vi "Quick Stacks.vi"(7 "Calling VI Ref":refnum<vi>) -> ()   [LabVIEW 2016]
uses:
  Hardware Configuration/Hardware Configuration Controls/Device Function.ctl
  Hardware Configuration/Hardware Configuration Controls/Device Type.ctl
  Quick Stacks Type Defs/Quick Stacks Notifier Type.ctl
  Quick Stacks Type Defs/Quick Stack Actions.ctl
  <vilib>/Utility/miscctls.llb/LVPointTypeDef.ctl
  Device Library/Stages/Stages Controls/Stage Actions.ctl
  Color Steps/Color Steps Type Def/Color Step Actions.ctl
  Tools/TIFF Image Read and Write/ImageJ TIF Type Defs/TIF Write Image Information.ctl
  Device Library/Cameras/Camera Controls/Generic Camera Actions.ctl
  Laser Control/Laser Power Control/Laser Power Control Type Defs/Laser Power Ctrl Messenger Actions.ctl
  shell32.dll
panel:
  in  "Camera 02":bool=TRUE
  in  "Camera 01":bool=TRUE
  out "Current Cycle":u16
  out "Current Step":u16
  in  "Start":bool
  in  "Number of Cycles":u16=1 min=1
  in  "Cycle Delay (s)":u32
  in  "Frames Per Step":u16=1 min=1
  in  "Base Save Path":path
  in  "File Name":string="Test Image"
  out "Z Range (µm)":dbl
  in  "Number of Steps":u16=1
  out "Step Size (µm)":dbl format="%#_3g"
  out "End Position (µm)":dbl
  out "Start Position (µm)":dbl
  in  "Set Z End":bool
  in  "Set Z Start":bool
  in  "Quit":bool
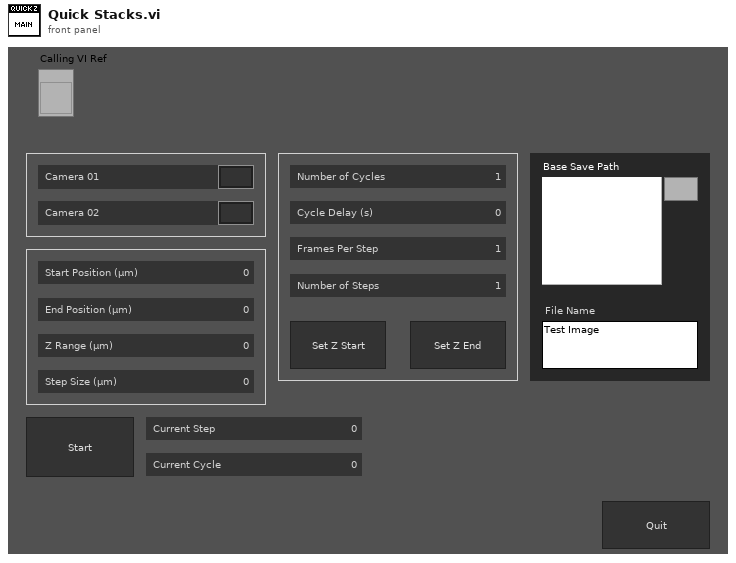
[diagram p1: front panel]
types:
  T1 = enum16{"Always On", "Always Off", "Off While Running"}
  T2 = typedef "LVPointTypeDef.ctl" = cluster{"Horizontal":i16, "Vertical":i16}
  T3 = typedef "Quick Stack Actions.ctl" = enum16{"Idle", "Update Range", "Start Acquisition", "Initial C Step", "Open File", "Close File", "Start Camera", "Stop Camera", "Laser On", "Laser Off", "Get Image", "Step Z", "Move to Z Start", "Step Color", "Check Cycle", "Abort", "Exit Loop", "Quit"}
  T4 = typedef "Quick Stacks Notifier Type.ctl" = cluster{"Actions":T3, "Start Z (µm)":dbl, "End Z (µm)":dbl, "Z Size (µm)":dbl, "Num of Steps":u16, "Frames per Step":u16, "Cycle Delay (s)":u32, "Num of Cycles":u16, "Save Path":path, "Running?":bool, "Save File Refs":refnum<file>[]}
  T5 = typedef "Device Function.ctl" = enum16{"Primary", "Secondary", "Overview", "Wide Field Drift Correction", "642 nm Excitation", "560 nm Excitation", "940 nm Excitation", "546 nm Excitation", "488 nm Excitation", "405 nm Excitation", "Objective Drift Correction", "4Pi Objective Lock", "Objective XY", "Objective Z", "Sample XY", "Sample Coarse Z", "Sample Z", "4Pi Lower", "4Pi Upper", "Mojo", "Adj Cavity", "Line Scanning", "Alert"}
  T6 = typedef "Device Type.ctl" = enum16{"AOTF", "Camera", "Deformable Mirror", "Laser", "Shutter", "Stage", "Waveform", "FPGA", "Email", "Filter Wheel"}
  T7 = typedef "LVRectTypeDef.ctl" = cluster{"Left":i16, "Top":i16, "Right":i16, "Bottom":i16}
  T8 = typedef "LVBoundsTypeDef.ctl" = cluster{"Width":u32, "Height":u32}
  T9 = typedef "Stage Actions.ctl" = enum16{"Get Position", "MVR", "MOVE", "HALT", "ONTARGET", "ERROR", "REFERENCE", "INIT", "VELOCITY", "STATUS", "EXIT", "HOME", "ZEROPOS", "NANOPOS", "ANALOG", "QUIT"}
  T10 = typedef "Color Step Actions.ctl" = enum16{"Add Step", "Update Step", "Remove Step", "Clear All", "Get Status", "Next Step", "Go To Step", "Save Preset", "Change Preset", "Update Names", "Quit"}
  T11 = typedef "Generic Camera Actions.ctl" = enum16{"Status", "Live Preview", "Capture", "Abort", "Set Exposure Time (s)", "Get Exposure Time (s)", "Record Settings", "Set ROI", "Get ROI", "Defect Correction On/Off", "Cooler On/Off", "Fan On/Off", "Quti"}
  T12 = typedef "TIF Write Image Information.ctl" = cluster{"Image Width (Pixels)":u32, "Image Height (Pixels)":u32, "Pixel Width (µm)":dbl, "Pixel Height (µm)":dbl, "Bits Per Sample (e.g. 16)":u32, "No. of Frames":u32, "No. of Slices":u32, "Time Step (sec)":dbl, "Z Step (µm)":dbl}
  T13 = typedef "Laser Power Ctrl Messenger Actions.ctl" = enum16{"All Active On", "All Off", "Adjust Power", "Line On/Off", "Get Status"}
  T14 = typedef "IMAQ Image.ctl" = refnum<image>
  T15 = typedef "Camera IMAQ Key Info.ctl" = cluster{"Frame":u32, "Sensor Height":i32, "Sensor Width":i32, "ROI Height":i32, "ROI Width":i32, "ROI Enable?":bool, "Bit per Pixel":u8}
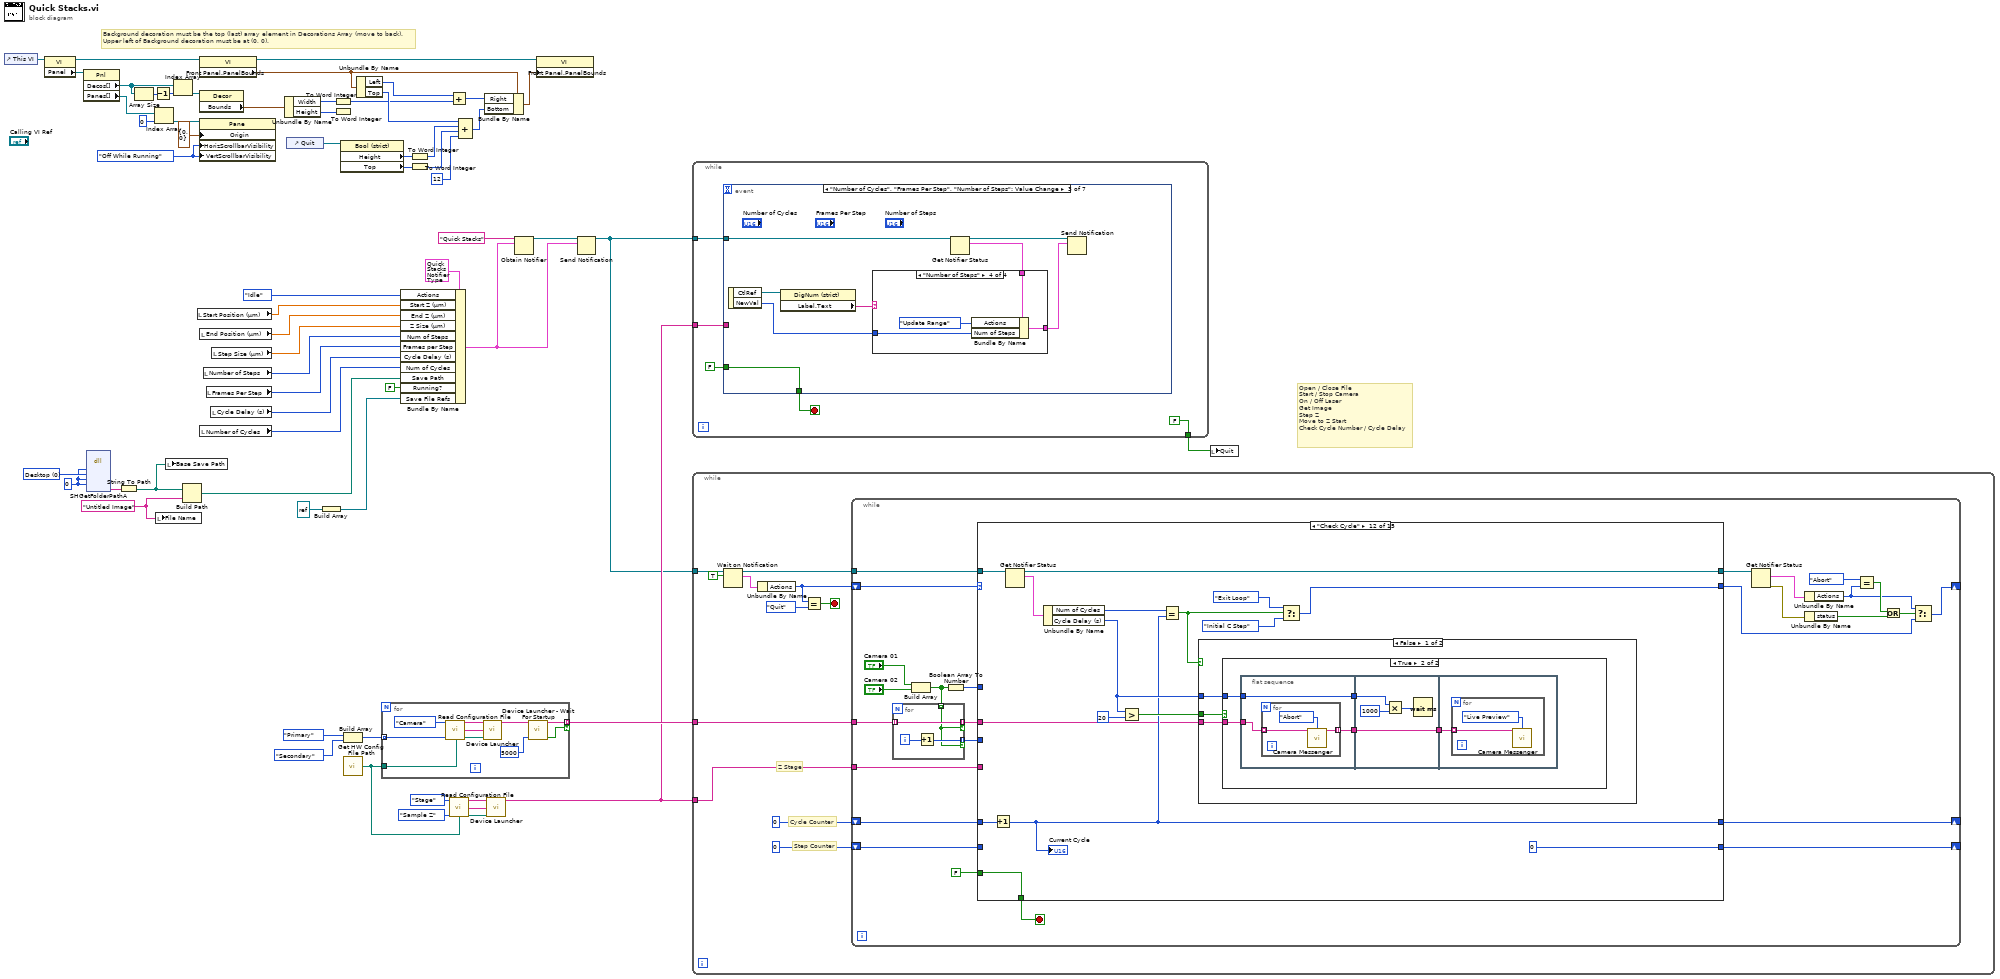
[diagram p0: block diagram]
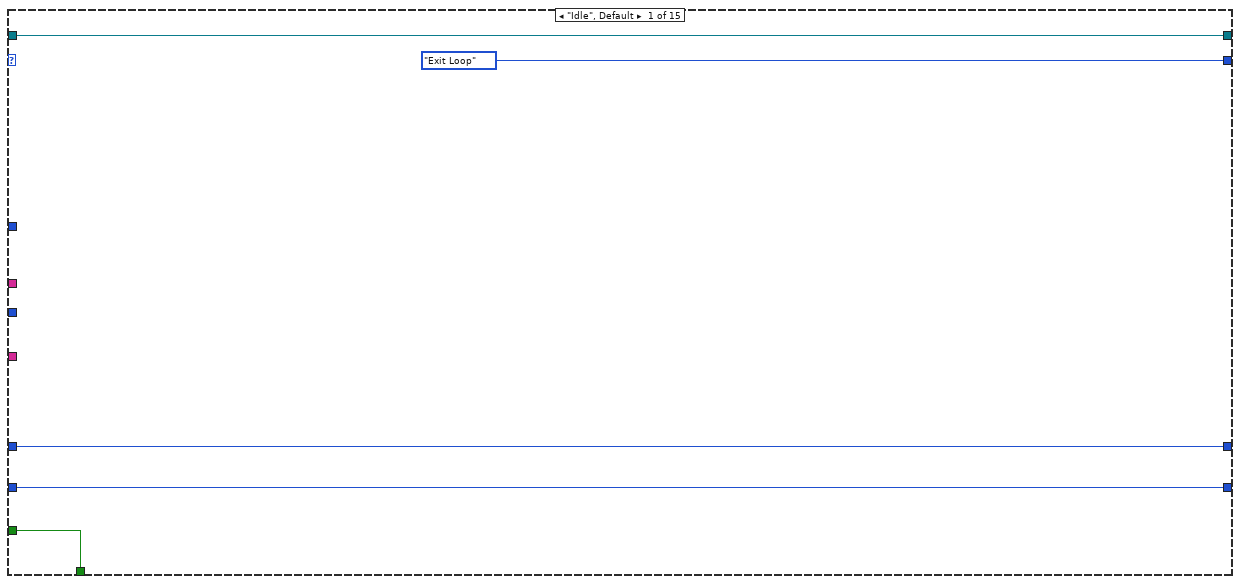
[diagram p2: hidden frame]
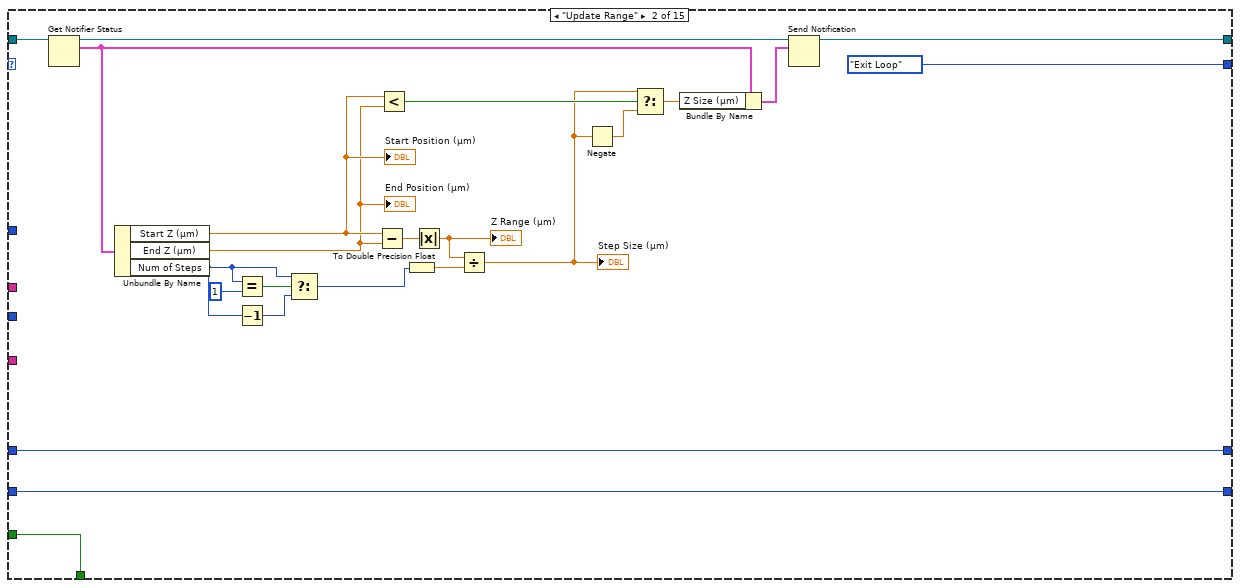
[diagram p3: hidden frame]
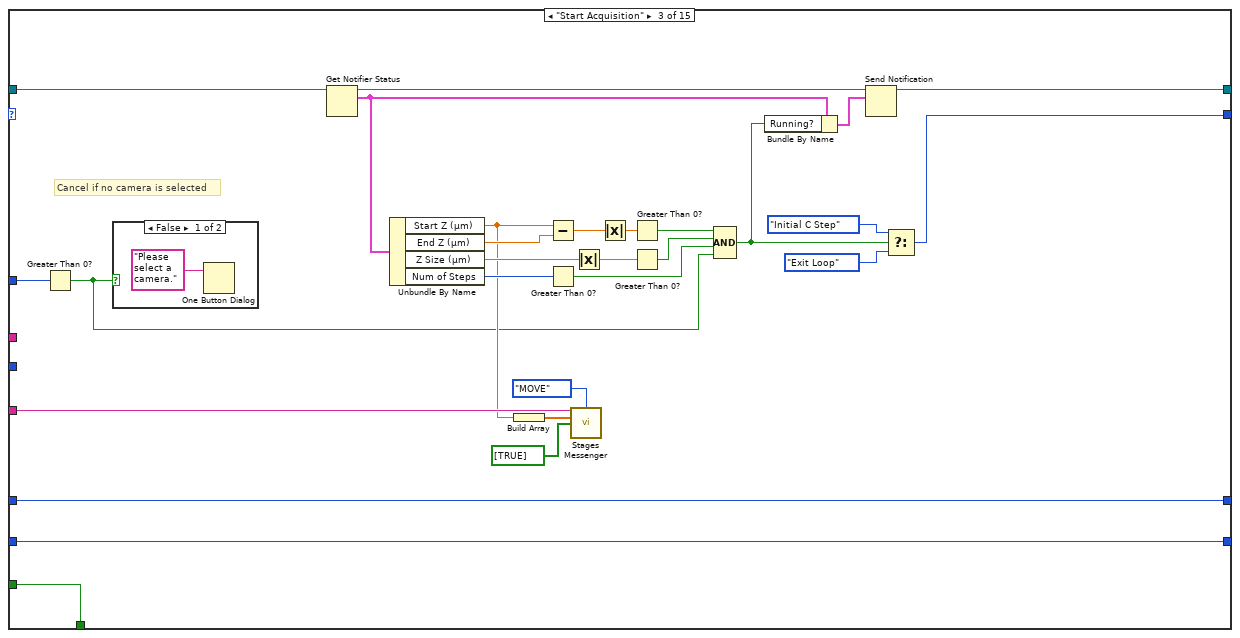
[diagram p4: hidden frame]
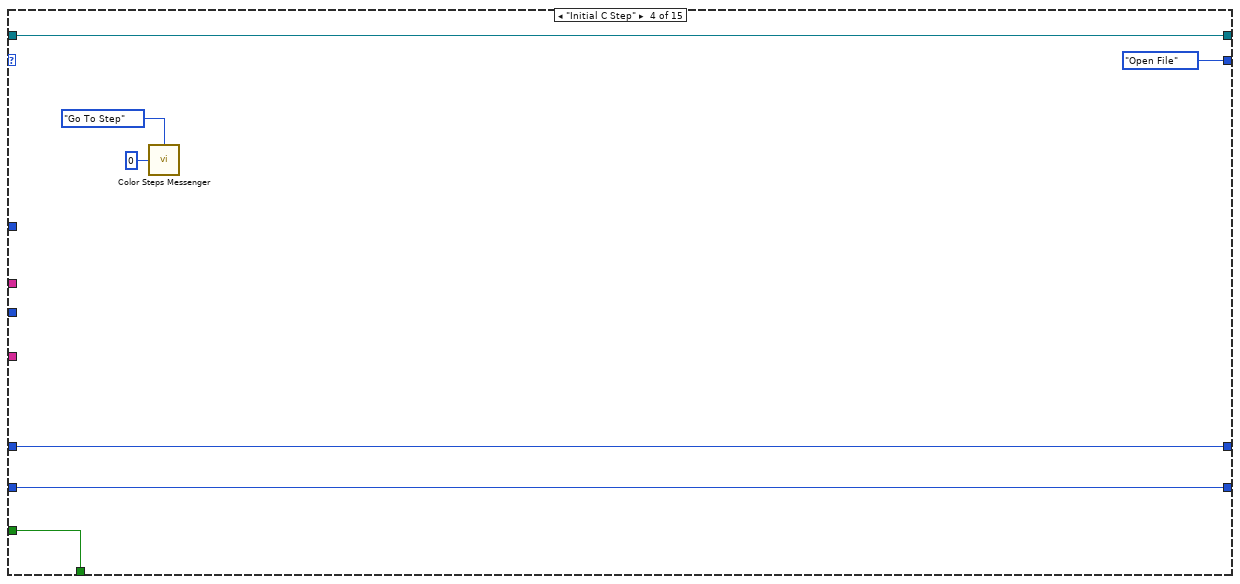
[diagram p6: hidden frame]
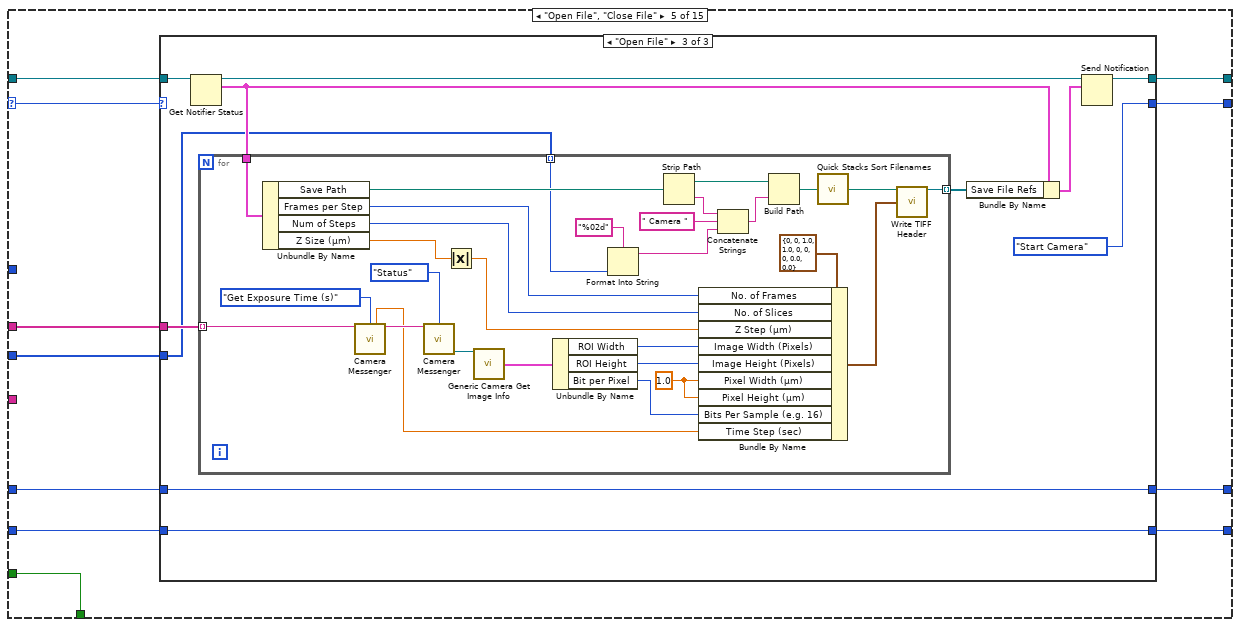
[diagram p7: hidden frame]
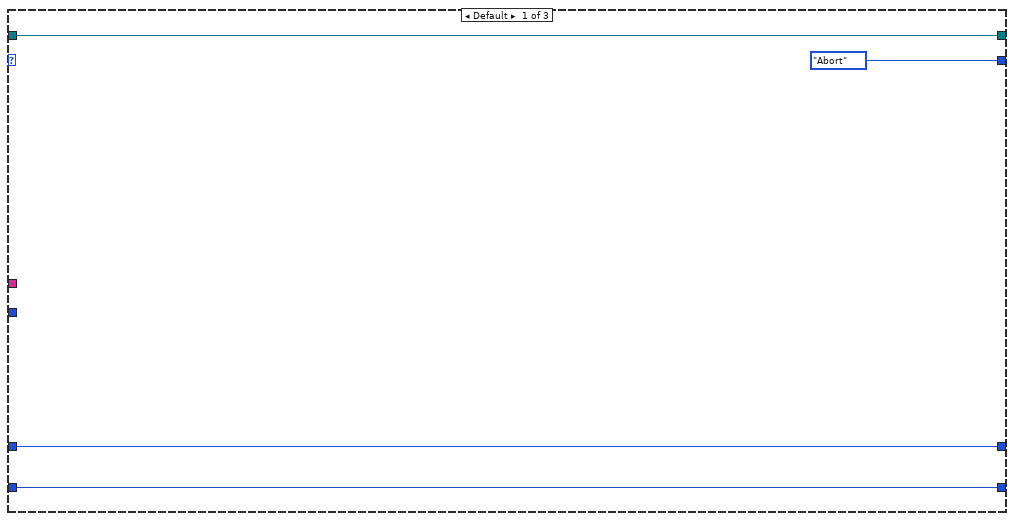
[diagram p8: hidden frame]
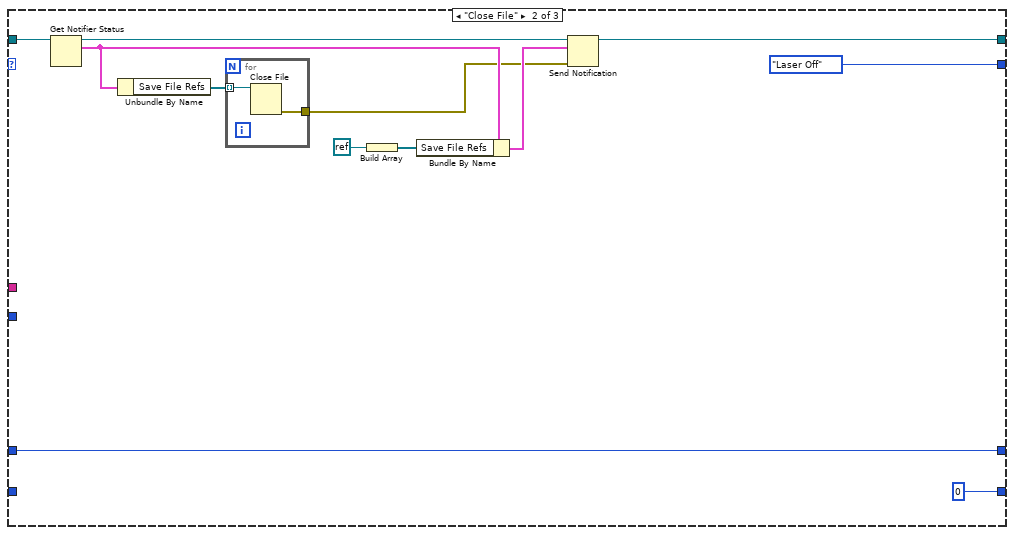
[diagram p9: hidden frame]
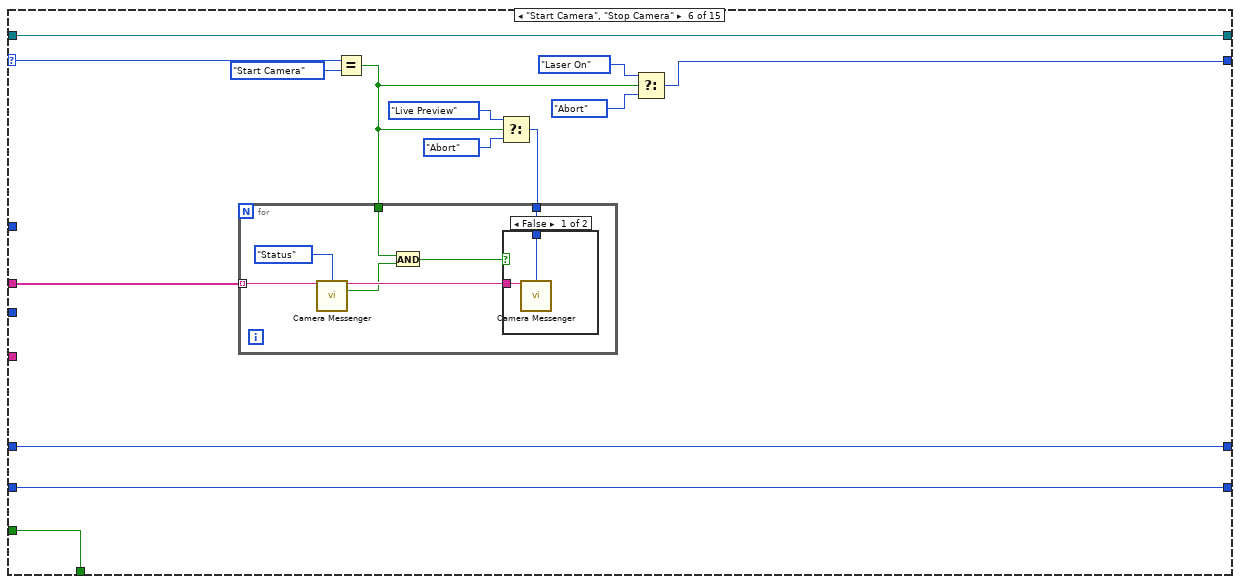
[diagram p10: hidden frame]
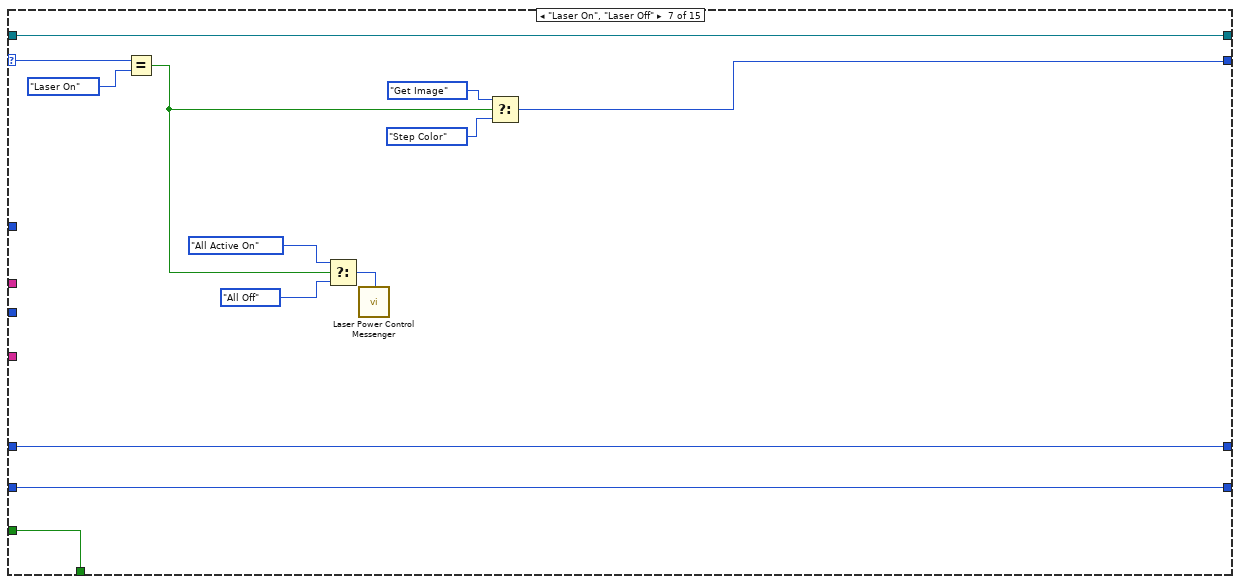
[diagram p12: hidden frame]
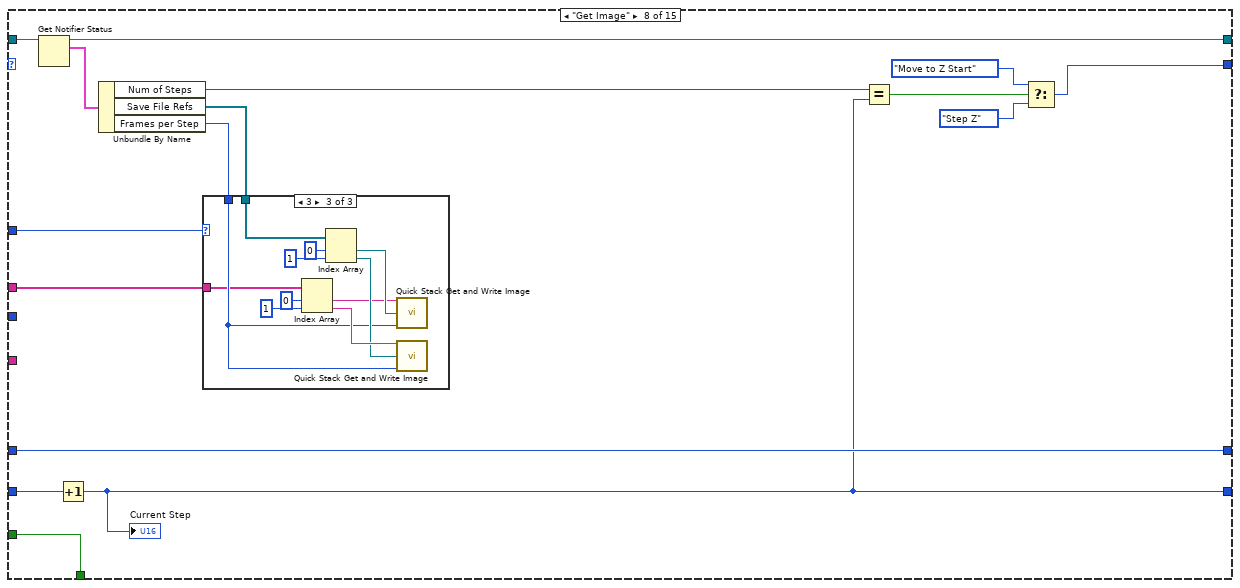
[diagram p13: hidden frame]
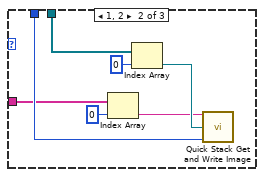
[diagram p15: hidden frame]
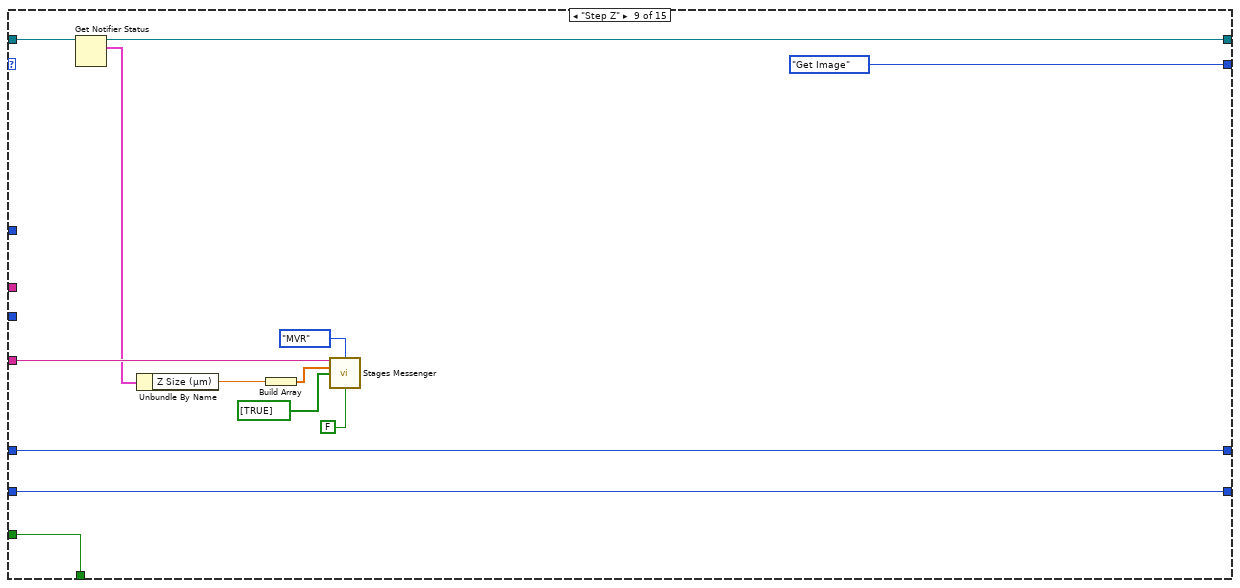
[diagram p16: hidden frame]
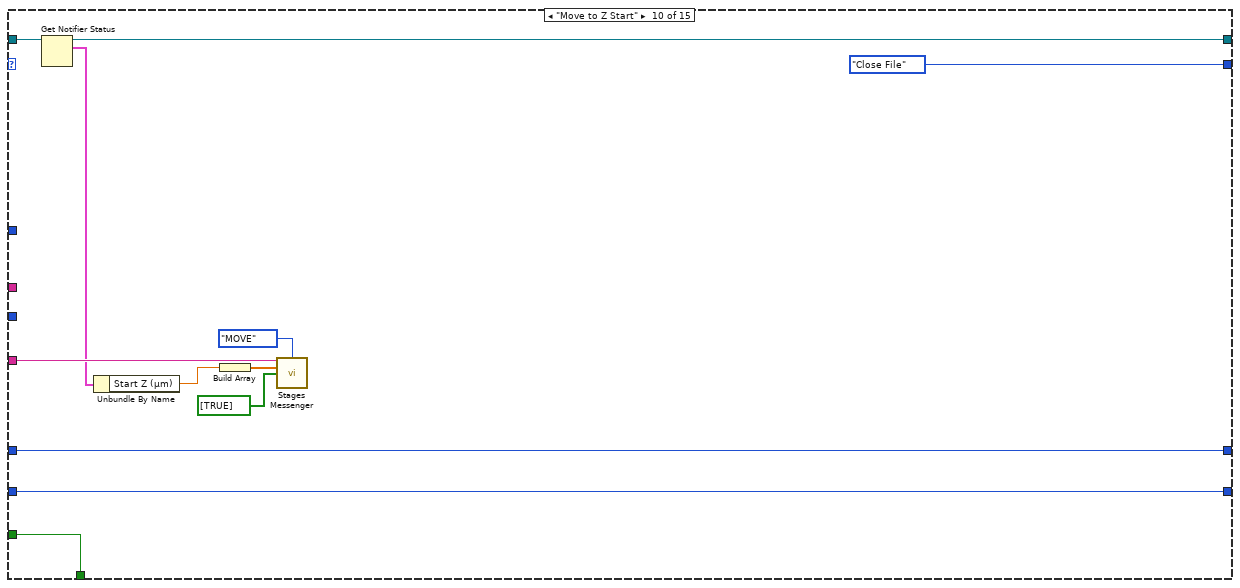
[diagram p17: hidden frame]
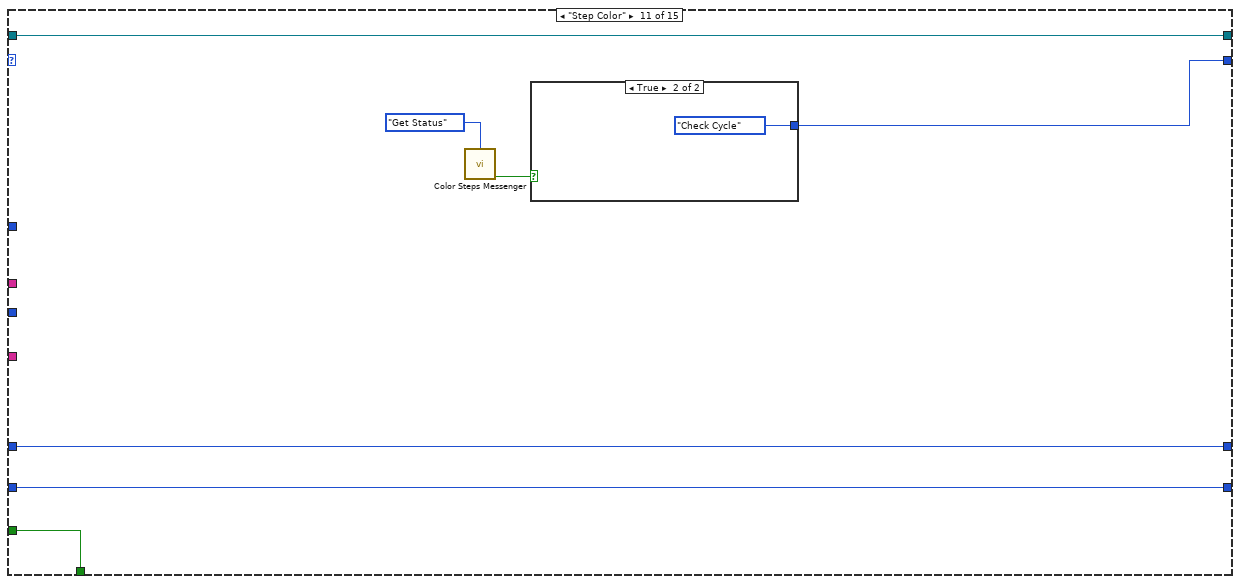
[diagram p18: hidden frame]
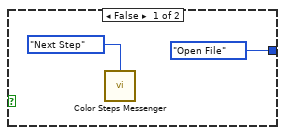
[diagram p19: hidden frame]
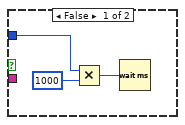
[diagram p20: hidden frame]
diagram:
  w15 = T1."Off While Running" ("Vertical Scrollbar Visibility")
  w49 = "Untitled Image"
  w52 = 0 items=["Desktop"=0, "Personal Documents"=5, "AppData"=26, "Local AppData"=28, "Common AppData"=35, "Program Files"=38, "Program Files Common"=43, "Common Documents"=46] ("Requested Path")
  w51 = 0 ("HWND")
  # "Background decoration must be the top (last) array element in Decorations Array (move to back).\nUpper left of Background decoration must be at (0, 0)."
  # "Open / Close File\nStart / Stop Camera\nOn / Off Laser\nGet Image\nStep Z\nMove to Z Start\nCheck Cycle Number / Cycle Delay"
  n1 = control-ref of="This VI"() -> (w7:refnum<vi>)
  n2 = property class="VI"(reference=w7) -> (reference out=w16:refnum<vi>, "Panel"=w8:refnum<vi>)  [unwired: 1 in, 1 out]
  n3 = property class="Pnl"(reference=w8) -> ("Decos[]"=w6:refnum<vi>[], "Panes[]"=w12:refnum<vi>[])  [unwired: 1 in, 2 out]
  n4 = dll-call lib="shell32.dll" fn="SHGetFolderPathA"("HWND"=w51, "nFolder"=w52, "hToken"=w51, "dwFlags"=w51) -> ("pszPath"=w50:string)  [unwired: 9 in, 2 out]
  n5 = String To Path(string=w50) -> (path=w48:path)
  n6 = Array Size(array=w6) -> (size(s)=w4:i32)
  n7 = Decrement(x=w4) -> (x-1=w5:i32)
  n8 = Index Array(array=w12, index=0) -> (element=w11:refnum<vi>)
  n9 = local write "File Name"(w49) -> ()
  n10 = local write "Base Save Path"(w48) -> ()
  n11 = Index Array(array=w6, index=w5) -> (element=w14:refnum<vi>)
  n12 = Build Path(base path=w48, name or relative path=w49) -> (appended path=w38:path)
  n13 = local read "Start Position (µm)"() -> (w39:dbl)
  n14 = property class="VI"(reference=w16) -> (reference out=w18:refnum<vi>, "Front Panel.PanelBounds"=w19:T7)  [unwired: 1 in, 1 out]
  n15 = property class="Decor"(reference=w14) -> ("Bounds"=w17:T8)  [unwired: 1 in, 2 out]
  n16 = property class="Pane"(reference=w11, "Origin"=T2 {"Horizontal"=0, "Vertical"=0}, "HorizScrollbarVisibility"=w15, "VertScrollbarVisibility"=w15) -> ()  [unwired: 1 in, 2 out]
  n17 = local read "End Position (µm)"() -> (w40:dbl)
  n18 = local read "Number of Cycles"() -> (w45:u16)
  n19 = local read "Number of Steps"() -> (w42:u16)
  n20 = local read "Frames Per Step"() -> (w43:u16)
  n21 = local read "Cycle Delay (s)"() -> (w44:u32)
  n22 = local read "Step Size (µm)"() -> (w41:dbl)
  n23 = Unbundle By Name(w17) -> ("Width"=w22:u32, "Height"=w25:u32)
  n24 = control-ref of="Quit"() -> (w9:refnum<vi>)
  n25 = Build Array(refnum<file> refnum ("Save File Ref")) -> (w1:refnum<file>[])
  n26 = To Word Integer(number=w22) -> (16bit integer=w24:i16)
  n27 = To Word Integer(number=w25) -> ()  [unwired: 1 out]
  n28 = property class="Bool (strict)"(reference=w9) -> ("Height"=w27:u32, "Top"=w28:i32)  [unwired: 1 in, 2 out]
  n29 = Build Array(Device_Function."Primary" ("Device Function"), Device_Function."Secondary" ("Device Function")) -> (w61:T5[])
  n30 = call "Get HW Config File Path.vi"() -> ("File Path"=w53:path)  [unwired: 14 in, 1 out]
  n31 = Unbundle By Name(w19) -> ("Left"=w21:i16, "Top"=w32:i16)
  n32 = for {
    tunnel: w61 -> [w69] mode=indexing
    tunnel: w53 -> [w68]
    tunnel: [w66] -> w54 mode=indexing if=w65
    n33 = call "Read Configuration File.vi"("Device Type"=Device_Type."Camera", "Device Function"=w69, "Config File Path"=w68) -> ("Unique Notifier Name"=w71:string, "Device Ports/IDs/Channels"=w73:string[], "Device Engine Path"=w72:path)  [unwired: 9 in, 1 out]
    n34 = call "Device Launcher.vi"("Notifier Name"=w71, "Device Ports/IDs/Channels"=w73, "Device Engine Path"=w72) -> ("Notifier Name"=w67:string)  [unwired: 11 in, 1 out]
    n35 = call "Device Launcher - Wait For Startup.vi"("Notifier Name"=w67, "Wait Time (ms)"=5000) -> ("Notifier Name (Dup)"=w66:string, "Running?"=w65:bool)  [unwired: 12 in]
  }
  n36 = Bundle By Name(cluster=T4 {"Actions"=enum."Idle", "Start Z (µm)"=0.0, "End Z (µm)"=0.0, "Z Size (µm)"=0.0, "Num of Steps"=0, "Frames per Step"=0, "Cycle Delay (s)"=0, "Num of Cycles"=0, "Save Path"=path "", "Running?"=FALSE, "Save File Refs"=[]} ("Stack Parameters"), "Actions"=Quick_Stack_Actions."Idle", "Start Z (µm)"=w39, "End Z (µm)"=w40, "Z Size (µm)"=w41, "Num of Steps"=w42, "Frames per Step"=w43, "Cycle Delay (s)"=w44, "Num of Cycles"=w45, "Save Path"=w38, "Running?"=FALSE ("Running"), "Save File Refs"=w1) -> (w33:T4)
  n37 = To Word Integer(number=w27) -> (16bit integer=w30:i16)
  n38 = To Word Integer(number=w28) -> (16bit integer=w31:i16)
  n39 = call "Read Configuration File.vi"("Device Type"=Device_Type."Stage", "Device Function"=Device_Function."Sample Z", "Config File Path"=w53) -> ("Unique Notifier Name"=w56:string, "Device Ports/IDs/Channels"=w58:string[], "Device Engine Path"=w57:path)  [unwired: 9 in, 1 out]
  n40 = Add(x=w21, y=w24) -> (x+y=w23:i16)
  n41 = Compound Arithmetic op=ADD(w32, w30, w31, i16 12 ("y")) -> (w26:i16)
  n42 = Bundle By Name(cluster=w19, "Right"=w23, "Bottom"=w26) -> (w20:T7)
  n43 = call "Device Launcher.vi"("Notifier Name"=w56, "Device Ports/IDs/Channels"=w58, "Device Engine Path"=w57) -> ("Notifier Name"=w37:string)  [unwired: 11 in, 1 out]
  n44 = Obtain Notifier(name (unnamed)="Quick Stacks", notification data type=w33) -> (notifier out=w35:refnum<notifier>)  [unwired: 2 in, 2 out]
  n45 = property class="VI"(reference=w18, "Front Panel.PanelBounds"=w20) -> ()  [unwired: 1 in, 2 out]
  n46 = Send Notification(notification=w33, notifier=w35) -> (notifier out=w34:refnum<notifier>)  [unwired: 1 in, 1 out]
  n47 = while {
    tunnel: w34 -> [w84]
    tunnel: w54 -> [w74]
    tunnel: w37 -> [w77]
    stop <- w81 stop-if-true
    # "Z Stage"
    # "Step Counter"
    # "Cycle Counter"
    n48 = Wait on Notification(notifier=w84, ignore previous (F)=TRUE) -> (notifier out=w80:refnum<notifier>, notification=w79:T4)  [unwired: 2 in, 2 out]
    n49 = Unbundle By Name(w79) -> ("Actions"=w78:T3)
    n50 = Equal?(x=w78, y=Quick_Stack_Actions."Quit") -> (x = y?=w81:bool)
    n51 = while {
      tunnel: w80 -> [w110]
      shift-right: [w92] -> _
      shift-left: w78 -> [w109]
      tunnel: w77 -> [w106]
      shift-right: [w102] -> _
      shift-left: u16 0 -> [w105]
      shift-right: [w103] -> _
      shift-left: u16 0 -> [w104]
      tunnel: w74 -> [w88]
      stop <- w107 stop-if-true
      n52 = Build Array("Camera 01", "Camera 02") -> (w87:bool[])
      n53 = for {
        tunnel: w88 -> [w431] mode=indexing
        tunnel: [w431] -> w89 mode=indexing if=w428
        tunnel: w87 -> [w428] mode=indexing
        tunnel: [w429] -> w85 mode=indexing if=w428
        i -> [w430]
        n54 = Increment(x=w430) -> (x+1=w429:i32)
      }
      n55 = Boolean Array To Number(Boolean array=w87) -> (number=w86:u32)
      n56 = case shown="\"Check Cycle\"" w109 {
        selector: w109 -> [_ _ _ _ w183 w256 w278 _ _ _ _ _ _ _ _]
        tunnel: w110 -> [w113 w136 w165 w174 w184 w249 w271 w293 w325 w333 w344 w361 w406 w417 w423]
        tunnel: FALSE -> [w115 w137 w166 w172 w185 w257 w279 w295 w326 w335 w345 w364 w407 _ _]
        tunnel: [w115 w137 w166 w172 w185 w257 w279 w295 w326 w335 w345 w364 w407 TRUE TRUE] -> w107
        tunnel: [Quick_Stack_Actions."Exit Loop" ("y") Quick_Stack_Actions."Exit Loop" ("y") w154 Quick_Stack_Actions."Open File" ("y") w182 w250 w275 w287 Quick_Stack_Actions."Get Image" ("y") Quick_Stack_Actions."Close File" ("y") w339 w355 Quick_Stack_Actions."Exit Loop" ("y") Quick_Stack_Actions."Exit Loop" ("y") Quick_Stack_Actions."Quit" ("y")] -> w93
        tunnel: w106 -> [_ _ w151 _ _ _ _ _ w323 w334 _ _ w401 _ _]
        tunnel: w105 -> [w112 w122 w147 w171 w178 w248 w273 w290 w322 w329 w341 w363 _ w420 w425]
        tunnel: w104 -> [w111 w121 w146 w170 w176 w247 w272 w294 w321 w330 w340 _ _ w419 w424]
        tunnel: [w113 w123 w144 w174 w181 w249 w271 w291 w320 w328 w344 w359 w398 w415 w423] -> w101
        tunnel: [w111 w121 w146 w170 w175 w247 w272 w284 w321 w330 w340 u16 0 w400 w419 w424] -> w103
        tunnel: [w112 w122 w147 w171 w177 w248 w273 w290 w322 w329 w341 w350 w400 w420 w425] -> w102
        tunnel: w89 -> [_ _ _ _ w180 w244 _ w281 _ _ _ w349 w394 _ _]
        tunnel: w86 -> [_ _ w140 _ _ _ _ w280 _ _ _ _ _ _ _]
        tunnel: w85 -> [_ _ _ _ w179 _ _ _ _ _ _ _ _ _ _]
        frame "Idle", Default {
        }
        frame "Update Range" {
          n57 = Get Notifier Status(notifier=w136) -> (notifier out=w135:refnum<notifier>, current notification=w134:T4)  [unwired: 1 in, 3 out]
          n58 = Unbundle By Name(w134) -> ("Start Z (µm)"=w130:dbl, "End Z (µm)"=w129:dbl, "Num of Steps"=w132:u16)
          "Start Position (µm)" <- w130
          "End Position (µm)" <- w129
          n59 = Equal?(x=w132, y=u16 1) -> (x = y?=w117:bool)
          n60 = Decrement(x=w132) -> (x-1=w118:u16)
          n61 = Select(t=w132, s=w117, f=w118) -> (s? t:f=w119:u16)
          n62 = Subtract(x=w130, y=w129) -> (x-y=w133:dbl)
          n63 = Less?(x=w130, y=w129) -> (x < y?=w127:bool)
          n64 = To Double Precision Float(number=w119) -> (double precision float=w120:dbl)
          n65 = Absolute Value(x=w133) -> (abs(x)=w131:dbl)
          "Z Range (µm)" <- w131
          n66 = Divide(x=w131, y=w120) -> (x/y=w125:dbl)
          "Step Size (µm)" <- w125
          n67 = Negate(x=w125) -> (-x=w124:dbl)
          n68 = Select(t=w125, s=w127, f=w124) -> (s? t:f=w126:dbl)
          n69 = Bundle By Name(cluster=w134, "Z Size (µm)"=w126) -> (w128:T4)
          n70 = Send Notification(notification=w128, notifier=w135) -> (notifier out=w123:refnum<notifier>)  [unwired: 1 in, 1 out]
        }
        frame "Start Acquisition" {
          # "Cancel if no camera is selected"
          n71 = Greater Than 0?(x=w140) -> (x > 0?=w139:bool)
          n72 = case shown="False" w139 {
            frame False {
              n73 = One Button Dialog(message="Please select a camera.") -> ()  [unwired: 1 in, 1 out]
            }
            frame True {
            }
          }
          n74 = Get Notifier Status(notifier=w165) -> (notifier out=w145:refnum<notifier>, current notification=w143:T4)  [unwired: 1 in, 3 out]
          n75 = Unbundle By Name(w143) -> ("Start Z (µm)"=w150:dbl, "End Z (µm)"=w164:dbl, "Z Size (µm)"=w163:dbl, "Num of Steps"=w161:u16)
          n76 = Build Array(w150) -> (w149:dbl[])
          n77 = Subtract(x=w150, y=w164) -> (x-y=w162:dbl)
          n78 = Greater Than 0?(x=w161) -> (x > 0?=w156:bool)
          n79 = call "Stages Messenger.vi"("Stage Notifier Name"=w151, "Actions"=Stage_Actions."MOVE", "Setpoint"=w149, "Axis"=bool[] [TRUE]) -> ()  [unwired: 8 in, 4 out]
          n80 = Absolute Value(x=w163) -> (abs(x)=w159:dbl)
          n81 = Absolute Value(x=w162) -> (abs(x)=w160:dbl)
          n82 = Greater Than 0?(x=w160) -> (x > 0?=w158:bool)
          n83 = Greater Than 0?(x=w159) -> (x > 0?=w157:bool)
          n84 = Compound Arithmetic op=AND(w158, w157, w156, w139) -> (w141:bool)
          n85 = Bundle By Name(cluster=w143, "Running?"=w141) -> (w142:T4)
          n86 = Send Notification(notification=w142, notifier=w145) -> (notifier out=w144:refnum<notifier>)  [unwired: 1 in, 1 out]
          n87 = Select(t=Quick_Stack_Actions."Initial C Step", s=w141, f=Quick_Stack_Actions."Exit Loop" ("y")) -> (s? t:f=w154:T3)
        }
        frame "Initial C Step" {
          n88 = call "Color Steps Messenger.vi"("Action"=Color_Step_Actions."Go To Step", "Step"=0) -> ()  [unwired: 12 in, 2 out]
        }
        frame "Open File", "Close File" {
          n89 = case shown="\"Open File\"" w183 {
            tunnel: w184 -> [w189 w201 w214]
            tunnel: [Quick_Stack_Actions."Abort" ("y") Quick_Stack_Actions."Laser Off" ("y") Quick_Stack_Actions."Start Camera" ("y")] -> w182
            tunnel: [w189 w196 w208] -> w181
            tunnel: w180 -> [_ _ w207]
            tunnel: w179 -> [_ _ w206]
            tunnel: w178 -> [w187 w191 w205]
            tunnel: [w187 w191 w205] -> w177
            tunnel: w176 -> [w186 _ w204]
            tunnel: [w186 u16 0 w204] -> w175
            frame Default {
            }
            frame "Close File" {
              n90 = Get Notifier Status(notifier=w201) -> (notifier out=w200:refnum<notifier>, current notification=w198:T4)  [unwired: 1 in, 3 out]
              n91 = Unbundle By Name(w198) -> ("Save File Refs"=w192:refnum<file>[])
              n92 = for {
                tunnel: [w203] -> w197
                tunnel: w192 -> [w202] mode=indexing
                n93 = Close File(refnum=w202) -> (error out=w203:errorcluster)  [unwired: 1 in, 1 out]
              }
              n94 = Build Array(refnum<k0> refnum) -> (w193:refnum<k0>[])
              n95 = Bundle By Name(cluster=w198, "Save File Refs"=w193) -> (w199:T4)
              n96 = Send Notification(notification=w199, notifier=w200, error in (no error)=w197) -> (notifier out=w196:refnum<notifier>)  [unwired: 1 out]
            }
            frame "Open File" {
              n97 = Get Notifier Status(notifier=w214) -> (notifier out=w213:refnum<notifier>, current notification=w212:T4)  [unwired: 1 in, 3 out]
              n98 = for {
                tunnel: w212 -> [w226]
                tunnel: [w225] -> w210 mode=indexing
                tunnel: w207 -> [w224] mode=indexing
                tunnel: w206 -> [w215] mode=indexing
                w235 = 1.0 ("Pixel Width (µm)")
                n99 = Unbundle By Name(w226) -> ("Save Path"=w218:path, "Frames per Step"=w230:u16, "Num of Steps"=w229:u16, "Z Size (µm)"=w231:dbl)
                n100 = call "Camera Messenger.vi"("Notifier Name"=w224, "General Camera Actions"=Generic_Camera_Actions."Get Exposure Time (s)") -> ("Current Exposure Time (s)"=w227:dbl, "Notifier Name Dup"=w232:string)  [unwired: 8 in, 4 out]
                n101 = call "Camera Messenger.vi"("Notifier Name"=w232, "General Camera Actions"=Generic_Camera_Actions."Status") -> ("Image Ref"=w240:T14)  [unwired: 8 in, 5 out]
                n102 = Absolute Value(x=w231) -> (abs(x)=w228:dbl)
                n103 = call "Generic Camera Get Image Info.vi"("Image Ref"=w240) -> ("Camera Image Info"=w239:T15)  [unwired: 14 in]
                n104 = Unbundle By Name(w239) -> ("ROI Width"=w238:i32, "ROI Height"=w237:i32, "Bit per Pixel"=w236:u8)
                n105 = Format Into String(format string="%02d", w215) -> (resulting string=w216:string)  [unwired: 2 in, 1 out]
                n106 = Strip Path(path=w218) -> (stripped path=w220:path, name=w219:string)
                n107 = Bundle By Name(cluster=T12 {"Image Width (Pixels)"=0, "Image Height (Pixels)"=0, "Pixel Width (µm)"=1.0, "Pixel Height (µm)"=1.0, "Bits Per Sample (e.g. 16)"=0, "No. of Frames"=0, "No. of Slices"=0, "Time Step (sec)"=0.0, "Z Step (µm)"=0.0} ("Image Info"), "No. of Frames"=w230, "No. of Slices"=w229, "Z Step (µm)"=w228, "Image Width (Pixels)"=w238, "Image Height (Pixels)"=w237, "Pixel Width (µm)"=w235, "Pixel Height (µm)"=w235, "Bits Per Sample (e.g. 16)"=w236, "Time Step (sec)"=w227) -> (w241:T12)
                n108 = Concatenate Strings(w219, " Camera " ("string"), w216) -> (w221:string)
                n109 = Build Path(base path=w220, name or relative path=w221) -> (appended path=w217:path)
                n110 = call "Quick Stacks Sort Filenames.vi"("Requested File Path"=w217) -> ("Resulting File Path"=w243:path)  [unwired: 14 in]
                n111 = call "Write TIFF Header.vi"("File Path"=w243, "Image Info"=w241) -> ("File Ref"=w225:refnum<file>)  [unwired: 11 in, 2 out]
              }
              n112 = Bundle By Name(cluster=w212, "Save File Refs"=w210) -> (w211:T4)
              n113 = Send Notification(notification=w211, notifier=w213) -> (notifier out=w208:refnum<notifier>)  [unwired: 1 in, 1 out]
            }
          }
        }
        frame "Start Camera", "Stop Camera" {
          n114 = Equal?(x=w256, y=Quick_Stack_Actions."Start Camera") -> (x = y?=w245:bool)
          n115 = Select(t=Generic_Camera_Actions."Live Preview" ("General Camera Actions"), s=w245, f=Generic_Camera_Actions."Abort") -> (s? t:f=w252:T11)
          n116 = for {
            tunnel: w252 -> [w264]
            tunnel: w245 -> [w261]
            tunnel: w244 -> [w258] mode=indexing
            n117 = call "Camera Messenger.vi"("Notifier Name"=w258, "General Camera Actions"=Generic_Camera_Actions."Status") -> ("Notifier Name Dup"=w262:string, "Running?"=w260:bool)  [unwired: 8 in, 4 out]
            n118 = And(x=w261, y=w260) -> (x .and. y?=w259:bool)
            n119 = case shown="False" w259 {
              tunnel: w264 -> [w266 _]
              tunnel: w262 -> [w265 _]
              frame False {
                n120 = call "Camera Messenger.vi"("Notifier Name"=w265, "General Camera Actions"=w266) -> ()  [unwired: 8 in, 6 out]
              }
              frame True {
              }
            }
          }
          n121 = Select(t=Quick_Stack_Actions."Laser On" ("y"), s=w245, f=Quick_Stack_Actions."Abort") -> (s? t:f=w250:T3)
        }
        frame "Laser On", "Laser Off" {
          n122 = Equal?(x=w278, y=Quick_Stack_Actions."Laser On") -> (x = y?=w267:bool)
          n123 = Select(t=Laser_Power_Ctrl_Messenger_Actions."All Active On" ("Power Ctrl Actions"), s=w267, f=Laser_Power_Ctrl_Messenger_Actions."All Off" ("Power Ctrl Actions")) -> (s? t:f=w268:T13)
          n124 = call "Laser Power Control Messenger.vi"("Power Ctrl Actions"=w268) -> ()  [unwired: 13 in, 2 out]
          n125 = Select(t=Quick_Stack_Actions."Get Image" ("y"), s=w267, f=Quick_Stack_Actions."Step Color") -> (s? t:f=w275:T3)
        }
        frame "Get Image" {
          n126 = Get Notifier Status(notifier=w293) -> (notifier out=w291:refnum<notifier>, current notification=w292:T4)  [unwired: 1 in, 3 out]
          n127 = Increment(x=w294) -> (x+1=w284:u16)
          "Current Step" <- w284
          n128 = Unbundle By Name(w292) -> ("Num of Steps"=w286:u16, "Save File Refs"=w283:refnum<file>[], "Frames per Step"=w282:u16)
          n129 = case shown="3" w280 {
            tunnel: w283 -> [_ w300 w308]
            tunnel: w282 -> [_ w298 w305]
            tunnel: w281 -> [_ w297 w304]
            frame 0, Default {
            }
            frame 1, 2 {
              n130 = Index Array(array=w297, index=0) -> (element=w296:string)
              n131 = Index Array(array=w300, index=0) -> (element=w299:refnum<file>)
              n132 = call "Quick Stack Get and Write Image.vi"("Notifier Name"=w296, "Write File Ref"=w299, "Num of Frames"=w298) -> ()  [unwired: 13 in]
            }
            frame 3 {
              n133 = Index Array(array=w304, index #1=0 ("index"), index #2=1 ("index")) -> (element #1=w303:string, element #2=w311:string)
              n134 = Index Array(array=w308, index #1=0 ("index"), index #2=1 ("index")) -> (element #1=w306:refnum<file>, element #2=w307:refnum<file>)
              n135 = call "Quick Stack Get and Write Image.vi"("Notifier Name"=w303, "Write File Ref"=w306, "Num of Frames"=w305) -> ()  [unwired: 13 in]
              n136 = call "Quick Stack Get and Write Image.vi"("Notifier Name"=w311, "Write File Ref"=w307, "Num of Frames"=w305) -> ()  [unwired: 13 in]
            }
          }
          n137 = Equal?(x=w286, y=w284) -> (x = y?=w289:bool)
          n138 = Select(t=Quick_Stack_Actions."Move to Z Start", s=w289, f=Quick_Stack_Actions."Step Z" ("y")) -> (s? t:f=w287:T3)
        }
        frame "Step Z" {
          n139 = Get Notifier Status(notifier=w325) -> (notifier out=w320:refnum<notifier>, current notification=w317:T4)  [unwired: 1 in, 3 out]
          n140 = Unbundle By Name(w317) -> ("Z Size (µm)"=w318:dbl)
          n141 = Build Array(w318) -> (w316:dbl[])
          n142 = call "Stages Messenger.vi"("Stage Notifier Name"=w323, "Actions"=Stage_Actions."MVR", "Setpoint"=w316, "Axis"=bool[] [TRUE], "Exit While Busy?"=FALSE) -> ()  [unwired: 7 in, 4 out]
        }
        frame "Move to Z Start" {
          n143 = Get Notifier Status(notifier=w333) -> (notifier out=w328:refnum<notifier>, current notification=w332:T4)  [unwired: 1 in, 3 out]
          n144 = Unbundle By Name(w332) -> ("Start Z (µm)"=w331:dbl)
          n145 = Build Array(w331) -> (w336:dbl[])
          n146 = call "Stages Messenger.vi"("Stage Notifier Name"=w334, "Actions"=Stage_Actions."MOVE", "Setpoint"=w336, "Axis"=bool[] [TRUE]) -> ()  [unwired: 8 in, 4 out]
        }
        frame "Step Color" {
          n147 = call "Color Steps Messenger.vi"("Action"=Color_Step_Actions."Get Status") -> ("Last Step"=w342:bool)  [unwired: 13 in, 1 out]
          n148 = case shown="True" w342 {
            tunnel: [Quick_Stack_Actions."Open File" ("y") Quick_Stack_Actions."Check Cycle" ("y")] -> w339
            frame False {
              n149 = call "Color Steps Messenger.vi"("Action"=Color_Step_Actions."Next Step") -> ()  [unwired: 13 in, 2 out]
            }
            frame True {
            }
          }
        }
        frame "Check Cycle" {
          n150 = Increment(x=w363) -> (x+1=w350:u16)
          "Current Cycle" <- w350
          n151 = Get Notifier Status(notifier=w361) -> (notifier out=w359:refnum<notifier>, current notification=w362:T4)  [unwired: 1 in, 3 out]
          n152 = Unbundle By Name(w362) -> ("Num of Cycles"=w360:u16, "Cycle Delay (s)"=w353:u32)
          n153 = Greater?(x=w353, y=u32 20) -> (0:w351:bool)
          n154 = Equal?(x=w360, y=w350) -> (x = y?=w358:bool)
          n155 = case shown="False" w358 {
            tunnel: w353 -> [w366 _]
            tunnel: w351 -> [w367 _]
            tunnel: w349 -> [w365 w389]
            frame False {
              n156 = case shown="True" w367 {
                tunnel: w366 -> [w368 w374]
                tunnel: w365 -> [_ w371]
                frame False {
                  n157 = Multiply(x=w368, y=u32 1000) -> (x*y=w369:u32)
                  n158 = Wait (ms)(milliseconds to wait=w369) -> ()  [unwired: 1 out]
                }
                frame True {
                  n159 = flat-sequence {
                    tunnel: [w378] -> w375
                    tunnel: w374 -> [w378]
                    tunnel: [w376] -> w372
                    tunnel: w371 -> [w377]
                    tunnel: w375 -> [w383]
                    tunnel: [w382] -> w373
                    tunnel: w372 -> [w382]
                    tunnel: w373 -> [w386]
                    frame #0 {
                      n160 = for {
                        tunnel: w377 -> [w380] mode=indexing
                        tunnel: [w379] -> w376 mode=indexing
                        n161 = call "Camera Messenger.vi"("Notifier Name"=w380, "General Camera Actions"=Generic_Camera_Actions."Abort") -> ("Notifier Name Dup"=w379:string)  [unwired: 8 in, 5 out]
                      }
                    }
                    frame #1 {
                      n162 = Multiply(x=w383, y=u32 1000) -> (x*y=w384:u32)
                      n163 = Wait (ms)(milliseconds to wait=w384) -> ()  [unwired: 1 out]
                    }
                    frame #2 {
                      n164 = for {
                        tunnel: w386 -> [w387] mode=indexing
                        n165 = call "Camera Messenger.vi"("Notifier Name"=w387, "General Camera Actions"=Generic_Camera_Actions."Live Preview") -> ()  [unwired: 8 in, 6 out]
                      }
                    }
                  }
                }
              }
            }
            frame True {
              n166 = for {
                tunnel: w389 -> [w390] mode=indexing
                n167 = call "Camera Messenger.vi"("Notifier Name"=w390, "General Camera Actions"=Generic_Camera_Actions."Abort") -> ()  [unwired: 8 in, 6 out]
              }
            }
          }
          n168 = Select(t=Quick_Stack_Actions."Exit Loop", s=w358, f=Quick_Stack_Actions."Initial C Step" ("y")) -> (s? t:f=w355:T3)
        }
        frame "Abort" {
          w400 = u16 0
          n169 = for {
            tunnel: w394 -> [w410] mode=indexing
            n170 = call "Camera Messenger.vi"("Notifier Name"=w410, "General Camera Actions"=Generic_Camera_Actions."Abort") -> ()  [unwired: 8 in, 6 out]
          }
          n171 = Get Notifier Status(notifier=w406) -> (notifier out=w399:refnum<notifier>, current notification=w397:T4)  [unwired: 1 in, 3 out]
          n172 = Unbundle By Name(w397) -> ("Save File Refs"=w393:refnum<file>[], "Start Z (µm)"=w402:dbl)
          n173 = call "Laser Power Control Messenger.vi"("Power Ctrl Actions"=Laser_Power_Ctrl_Messenger_Actions."All Off") -> ()  [unwired: 13 in, 2 out]
          n174 = Bundle By Name(cluster=w397, "Actions"=Quick_Stack_Actions."Exit Loop") -> (w395:T4)
          n175 = Build Array(w402) -> (w403:dbl[])
          n176 = for {
            tunnel: w393 -> [w409] mode=indexing
            n177 = Close File(refnum=w409) -> ()  [unwired: 1 in, 2 out]
          }
          n178 = call "Stages Messenger.vi"("Stage Notifier Name"=w401, "Actions"=Stage_Actions."MOVE", "Setpoint"=w403, "Axis"=bool[] [TRUE]) -> ()  [unwired: 8 in, 4 out]
          n179 = Send Notification(notification=w395, notifier=w399) -> (notifier out=w398:refnum<notifier>)  [unwired: 1 in, 1 out]
        }
        frame "Exit Loop" {
          n180 = Get Notifier Status(notifier=w417) -> (notifier out=w416:refnum<notifier>, current notification=w414:T4)  [unwired: 1 in, 3 out]
          n181 = Bundle By Name(cluster=w414, "Running?"=FALSE ("Running")) -> (w412:T4)
          n182 = local write "Start"(FALSE ("Start")) -> ()
          n183 = Send Notification(notification=w412, notifier=w416) -> (notifier out=w415:refnum<notifier>)  [unwired: 1 in, 1 out]
        }
        frame "Quit" {
          n184 = Release Notifier(notifier=w423) -> ()  [unwired: 2 in, 3 out]
        }
      }
      n185 = Get Notifier Status(notifier=w101) -> (current notification=w100:T4, error out=w99:errorcluster)  [unwired: 1 in, 3 out]
      n186 = Unbundle By Name(w100) -> ("Actions"=w94:T3)
      n187 = Unbundle By Name(w99) -> ("status"=w97:bool)
      n188 = Equal?(x=Quick_Stack_Actions."Abort", y=w94) -> (x = y?=w96:bool)
      n189 = Or(x=w96, y=w97) -> (x .or. y?=w95:bool)
      n190 = Select(t=w94, s=w95, f=w93) -> (s? t:f=w92:T3)
    }
  }
  n191 = while {
    tunnel: w34 -> [w434]
    tunnel: w37 -> [w433]
    tunnel: [FALSE] -> w36
    stop <- w436 stop-if-true
    n192 = event shown="[2] \"Number of Cycles\", \"Frames Per Step\", \"Number of Steps\": Value Change" {
      selector: _ -> [_ _ _ _ _ _ _]
      dyn-events: _ -> [_ _ _ _ _ _ _]
      timeout: _ -> [_ _ _ _ _ _ _]
      tunnel: [w437 w449 w468 w490 w499 w508 w514] -> w436
      tunnel: FALSE -> [w437 w449 w468 w490 w499 w508 _]
      tunnel: w434 -> [_ w446 w465 w488 w497 w504 w513]
      tunnel: w433 -> [_ w445 _ _ _ _ _]
      event Timeout {
        n193 = event-data() -> ()  [unwired: 1 in, 3 out]
      }
      event "Set Z Start", "Set Z End": Value Change {
        n194 = event-data() -> ("CtlRef"=w448:refnum<vi>)  [unwired: 1 in]
        n195 = property class="Bool"(reference=w448) -> ("Label.Text"=w447:string)  [unwired: 1 in, 2 out]
        n196 = call "Stages Messenger.vi"("Stage Notifier Name"=w445, "Actions"=Stage_Actions."Get Position") -> ("Positions"=w443:dbl[])  [unwired: 10 in, 3 out]
        n197 = Index Array(array=w443, index=0) -> (element=w441:dbl)
        n198 = Get Notifier Status(notifier=w446) -> (notifier out=w440:refnum<notifier>, current notification=w439:T4)  [unwired: 1 in, 3 out]
        n199 = case shown="\"Set Z Start\"" w447 {
          tunnel: w441 -> [_ w455 w459]
          tunnel: w439 -> [w452 w456 w460]
          tunnel: [w450 w453 w457] -> w438
          frame Default {
            n200 = Bundle By Name(cluster=w452, "Actions"=Quick_Stack_Actions."Idle") -> (w450:T4)
          }
          frame "Set Z Start" {
            n201 = Bundle By Name(cluster=w456, "Actions"=Quick_Stack_Actions."Update Range", "Start Z (µm)"=w455) -> (w453:T4)
          }
          frame "Set Z End" {
            n202 = Bundle By Name(cluster=w460, "Actions"=Quick_Stack_Actions."Update Range", "End Z (µm)"=w459) -> (w457:T4)
          }
        }
        n203 = Send Notification(notification=w438, notifier=w440) -> ()  [unwired: 1 in, 2 out]
      }
      event "Number of Cycles", "Frames Per Step", "Number of Steps": Value Change {
        n204 = event-data() -> ("CtlRef"=w467:refnum<vi>, "NewVal"=w462:u16)  [unwired: 1 in]
        n205 = property class="DigNum (strict)"(reference=w467) -> ("Label.Text"=w464:string)  [unwired: 1 in, 2 out]
        n206 = Get Notifier Status(notifier=w465) -> (notifier out=w466:refnum<notifier>, current notification=w463:T4)  [unwired: 1 in, 3 out]
        n207 = case shown="\"Number of Steps\"" w464 {
          tunnel: w463 -> [w471 w475 w479 w483]
          tunnel: w462 -> [_ w473 w477 w481]
          tunnel: [w469 w472 w476 w480] -> w461
          frame Default {
            n208 = Bundle By Name(cluster=w471, "Actions"=Quick_Stack_Actions."Idle") -> (w469:T4)
          }
          frame "Number of Cycles" {
            n209 = Bundle By Name(cluster=w475, "Actions"=Quick_Stack_Actions."Idle", "Num of Cycles"=w473) -> (w472:T4)
          }
          frame "Frames Per Step" {
            n210 = Bundle By Name(cluster=w479, "Actions"=Quick_Stack_Actions."Idle", "Frames per Step"=w477) -> (w476:T4)
          }
          frame "Number of Steps" {
            n211 = Bundle By Name(cluster=w483, "Actions"=Quick_Stack_Actions."Update Range", "Num of Steps"=w481) -> (w480:T4)
          }
        }
        n212 = Send Notification(notification=w461, notifier=w466) -> ()  [unwired: 1 in, 2 out]
      }
      event "Cycle Delay (s)": Value Change {
        n213 = event-data() -> ("NewVal"=w486:u32)  [unwired: 1 in]
        n214 = Get Notifier Status(notifier=w488) -> (notifier out=w489:refnum<notifier>, current notification=w487:T4)  [unwired: 1 in, 3 out]
        n215 = Bundle By Name(cluster=w487, "Actions"=Quick_Stack_Actions."Idle", "Cycle Delay (s)"=w486) -> (w485:T4)
        n216 = Send Notification(notification=w485, notifier=w489) -> ()  [unwired: 1 in, 2 out]
      }
      event "Base Save Path", "File Name": Value Change {
        n217 = event-data() -> ()  [unwired: 1 in, 1 out]
        n218 = Build Path(base path="Base Save Path", name or relative path="File Name") -> (appended path=w491:path)
        n219 = Get Notifier Status(notifier=w497) -> (notifier out=w498:refnum<notifier>, current notification=w496:T4)  [unwired: 1 in, 3 out]
        n220 = Bundle By Name(cluster=w496, "Actions"=Quick_Stack_Actions."Idle", "Save Path"=w491) -> (w495:T4)
        n221 = Send Notification(notification=w495, notifier=w498) -> ()  [unwired: 1 in, 2 out]
      }
      event "Start": Value Change {
        n222 = event-data() -> ("NewVal"=w503:bool)  [unwired: 1 in]
        n223 = Select(t=Quick_Stack_Actions."Start Acquisition" ("Actions"), s=w503, f=Quick_Stack_Actions."Abort" ("Actions")) -> (s? t:f=w500:T3)
        n224 = Get Notifier Status(notifier=w504) -> (notifier out=w507:refnum<notifier>, current notification=w506:T4)  [unwired: 1 in, 3 out]
        n225 = Bundle By Name(cluster=w506, "Actions"=w500) -> (w505:T4)
        n226 = Send Notification(notification=w505, notifier=w507) -> ()  [unwired: 1 in, 2 out]
      }
      event "Quit": Value Change {
        n227 = event-data() -> ("NewVal"=w514:bool)  [unwired: 1 in]
        n228 = Get Notifier Status(notifier=w513) -> (notifier out=w510:refnum<notifier>, current notification=w512:T4)  [unwired: 1 in, 3 out]
        n229 = Bundle By Name(cluster=w512, "Actions"=Quick_Stack_Actions."Quit") -> (w509:T4)
        n230 = Send Notification(notification=w509, notifier=w510) -> ()  [unwired: 1 in, 2 out]
      }
    }
  }
  n231 = local write "Quit"(w36) -> ()
